vi "[ce low] Differentiation XX.vi"(0 "start":dbl format="%.6e", 1 "VC Handle":T2=-1, 2 "# points":u32=100, 5 "end":dbl=1.0 format="%.6e", 7 "include end point":bool, 9 "formula info":cluster{"formula":string, "x-variable":string}={"formula"="", "x-variable"="t"}, 11 "error in":errorcluster, 12 "h":dbl=1e-08 format="%.2e", 13 "vm cmd":T1(ring)) -> (4 "X Values":dbl[](array[numeric]) format="%.8e", 6 "Y Values":dbl[](array[numeric]) format="%.8e", 8 "Derivative of Y":dbl[](array[numeric]) format="%.8e", 10 "dx":dbl format="%.6e", 15 "error out":errorcluster)   [LabVIEW 2021]
doc: "::: CalcExpress Toolkit :::\nCopyright (c) 2000-2026 Konstantin Shifershteyn. All rights reserved."
uses:
  cetypes.llb/VarMan Variable Context Handle.ctl
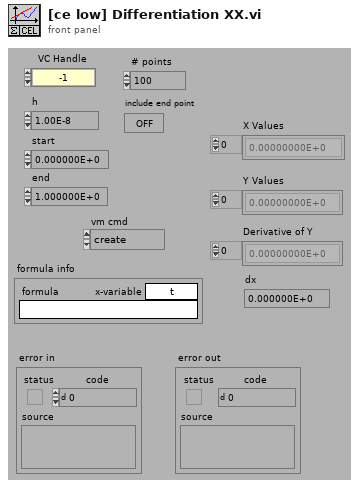
[diagram p1: front panel]
types:
  T1 = enum16{"create", "destroy", "set value", "get value"}
  T2 = typedef "VarMan Variable Context Handle.ctl" = i32
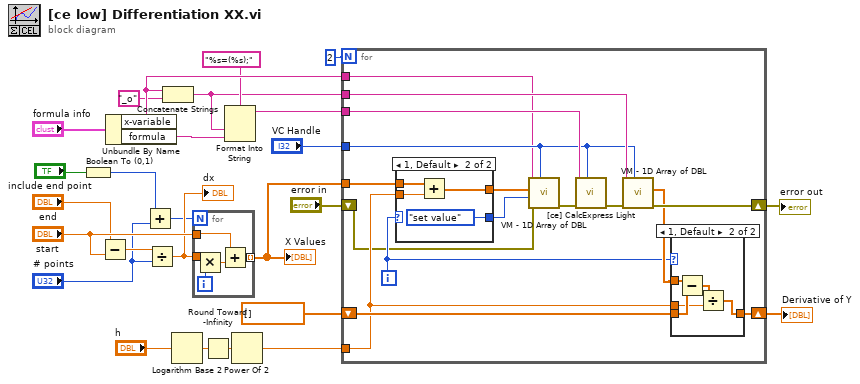
[diagram p0: block diagram]
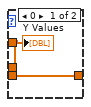
[diagram p2: hidden frame]
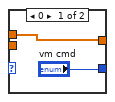
[diagram p3: hidden frame]
diagram:
  n1 = Boolean To (0,1)(Boolean="include end point") -> (0, 1=w1:i16)
  n2 = Subtract(x="end", y="start") -> (x-y=w18:dbl)
  n3 = Unbundle By Name("formula info") -> ("x-variable"=w25:string, "formula"=w11:string)
  n4 = Add(x=w1, y="# points") -> (x+y=w4:u32)
  n5 = Divide(x=w18, y="# points") -> (x/y=w6:dbl)
  "dx" <- w6
  n6 = Concatenate Strings(w25, "_o" ("Substring")) -> (w10:string)
  n7 = Logarithm Base 2(1:"h") -> (0:w15:dbl)
  n8 = for {
    N: w4 -> [_]
    tunnel: w6 -> [w31]
    tunnel: "start" -> [w28]
    tunnel: [w27] -> w5 mode=indexing
    i -> [w30]
    n9 = Multiply(x=w31, y=w30) -> (x*y=w29:dbl)
    n10 = Add(x=w28, y=w29) -> (x+y=w27:dbl)
  }
  "X Values" <- w5
  n11 = Round Toward -Infinity(1:w15) -> (0:w16:dbl)
  n12 = Format Into String(format string="%s=(%s);" ("Format String"), w10, w11) -> (resulting string=w9:string)  [unwired: 2 in, 1 out]
  n13 = Power Of 2(x=w16) -> (2^x=w24:dbl)
  n14 = for {
    N: 2 -> [_]
    shift-right: [w43] -> w26
    shift-left: "error in" -> [w35]
    tunnel: "VC Handle" -> [w37]
    tunnel: w9 -> [w46]
    tunnel: w10 -> [w45]
    tunnel: w25 -> [w34]
    tunnel: w5 -> [w44]
    shift-right: [w40] -> w22
    shift-left: dbl[] [] -> [w41]
    tunnel: w24 -> [w38]
    i -> [w39]
    n15 = case shown="1, Default" w39 {
      tunnel: w44 -> [w55 w59]
      tunnel: w38 -> [_ w58]
      tunnel: [w55 w57] -> w36
      tunnel: ["vm cmd" T1."set value" ("cmd")] -> w32
      frame 0 {
      }
      frame 1, Default {
        n16 = Add(x=w59, y=w58) -> (x+y=w57:dbl[])
      }
    }
    n17 = call "VM - 1D Array of DBL.vi"("VC Handle"=w37, "error in"=w35, "cmd"=w32, "value in"=w36, "name_spec"=w34) -> ("error out"=w33:errorcluster)  [unwired: 1 in, 5 out]
    n18 = call "[ce] CalcExpress Light.vi"("VC Handle"=w37, "error in"=w33, "expression"=w46) -> ("error out"=w47:errorcluster)  [unwired: 6 in, 2 out]
    n19 = call "VM - 1D Array of DBL.vi"("VC Handle"=w37, "error in"=w47, "name_spec"=w45) -> ("error out"=w43:errorcluster, "value out"=w42:dbl[])  [unwired: 3 in, 4 out]
    n20 = case shown="1, Default" w39 {
      tunnel: w42 -> [w48 w53]
      tunnel: w41 -> [_ w52]
      tunnel: [w48 w50] -> w40
      tunnel: w38 -> [_ w49]
      frame 0 {
        "Y Values" <- w48
      }
      frame 1, Default {
        n21 = Subtract(x=w53, y=w52) -> (x-y=w51:dbl[])
        n22 = Divide(x=w51, y=w49) -> (x/y=w50:dbl[])
      }
    }
  }
  "Derivative of Y" <- w22
  "error out" <- w26
